vi "Add New Line.vi"(8 "error in":errorcluster, 11 "objects":T1) -> (0 "error out":errorcluster, 1 "success":bool)   [LabVIEW 2015, in "Scan Engine editor node.lvclass"]
doc: "This VI is called to add new elements to the configuration. \nIt creates a new default line and the opens the dialog to edit its properties. \nFinally it adds it to the configuration."
uses:
  Scan Engine editor node.lvclass
  <vilib>/NI/DCAF/Tag Editor Core/Table API/Table Manager/object ref.ctl
  <vilib>/NI/DCAF/Tag Editor Core/Configuration Editor/Classes/Engine Parent/Engine Parent Editor Node.lvclass
  <vilib>/NI/DCAF/Tag Editor Core/Configuration Editor/Classes/Module editor node/module editor node.lvclass
  <vilib>/NI/DCAF/Tag Editor Core/Table API/Table Manager/Table Manager.lvclass
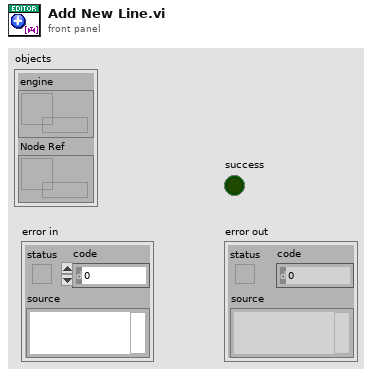
[diagram p1: front panel]
types:
  T1 = typedef "Table Manager.lvlib/Table Manager.lvclass/object ref.ctl" = cluster{"engine":refnum<data-value>, "Node Ref":refnum<data-value>}
  T2 = typedef "Scan Engine configuration.lvclass/Line.ctl" = cluster{"channel":refnum<class "TBM channel.lvclass">, "Tag":string}
  T3 = typedef "Scan Engine editor node.lvclass/Mappings.ctl" = cluster{"Line":T2, "Maps":T4[]}
  T4 = typedef "Scan Engine editor node.lvclass/Map.ctl" = cluster{"channel":refnum<class "TBM channel.lvclass">, "tag name":string}
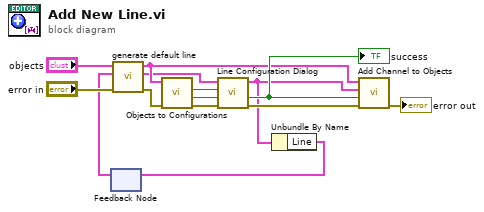
[diagram p0: block diagram]
diagram:
  n1 = feedback #1() -> (w3:T2)  [unwired: 1 in]
  n2 = call "generate default line.vi"("error in"="error in", "Last Line In"=w3, "objects in"="objects") -> ("error out"=w7:errorcluster, "Line out"=w4:T2, "objects out"=w9:T1)  [unwired: 6 in]
  n3 = call "Objects to Configurations.vi"("error in (no error)"=w7, "Objects in"=w9) -> ("error out"=w8:errorcluster, "engine configuration out"=w5:refnum<class "engine configuration.lvclass">, "tag bus configurable plugin module configuration"=w6:refnum<class "Scan Engine configuration.lvclass">)  [unwired: 7 in]
  n4 = call "Line Configuration Dialog.vi"("error in"=w8, "engine configuration in"=w5, "tag bus configurable plugin module configuration"=w6, "Line"=w4) -> ("error out"=w12:errorcluster, "success"=w10:bool, "Mappings out"=w2:T3)  [unwired: 4 in, 1 out]
  "success" <- w10
  n5 = Unbundle By Name(w2) -> ("Line"=w1:T2)
  n6 = feedback-in #1(w1) -> ()
  n7 = call "Add Channel to Objects.vi"("error in"=w12, "success"=w10, "line item in"=w2, "Objects in"=w9) -> ("error out"=→"error out":errorcluster)  [unwired: 7 in]
